vi "Test App Processes are Initialized.vi"(8 "error in (no error)":errorcluster, 11 "Rig Test In":refnum<class "Application Dev Test.lvclass">) -> (0 "error out":errorcluster, 3 "Rig Test Out":refnum<class "Application Dev Test.lvclass">)   [LabVIEW 2020, in "Application Dev Test.lvclass"]
uses:
  Application Dev Test.lvclass
  C:/Program Files (x86)/National Instruments/LabVIEW 2020/vi.lib/Astemes/LUnit/Test Case.lvclass
  source/Framework Test Suite/Mock Process/Mock Process.lvclass
  C:/Git/astemes-triarc-framework/source/Framework/Process/Process.lvclass
  source/Framework/Process/Process.lvclass/Process.ctl
  source/Framework/Application/Application.lvclass/Application.ctl
  <vilib>/Astemes/LUnit/Test Case.lvclass/Test Case.ctl
  source/Framework/Application/Private/Add Process to Map.vi
  source/Framework/Application/Private/Throw Error If Process Already in App.vi
  source/Framework/Process/Protected/Messaging/Send Message.vi
  source/Framework/Process/Public/Lifecycle/Get Lifecycle State.vi
  source/Framework/Process/Protected/SubVIs/Set Context.vi
  <vilib>/Astemes/LUnit/Palette/Fail.vi
  <vilib>/Astemes/LUnit/Palette/Pass.vi
  <vilib>/Astemes/LUnit/Set Assertion Type.vi
  source/Framework/Process/Protected/Messaging/Request Message.vi
  source/Framework/Process/Private/SubVIs/Wait for finish.vi
  source/Framework/Process/Private/SubVIs/Set Lifecycle State.vi
  source/Framework/Application/Public/Get Process.vi
  source/Framework/Process/Private/SubVIs/Handle Debug Data.vi
  <vilib>/Utility/error.llb/Clear Errors.vi
  source/Framework/Process/Public/Lifecycle/Leave Process Loop.vi
  <vilib>/Astemes/LUnit/Add test result.vi
  source/Framework/Process/Private/SubVIs/Enqueue Request Message.vi
  source/Framework/Application/Private/Retrieve Process from App.vi
  source/Framework/Application/Private/Parse Process Name.vi
  source/Framework/Application/Private/Get Process from Map.vi
  source/Framework/Logging/Log Debug.vi
  <vilib>/AdvancedString/1D String Array to Delimited String.vi
  <vilib>/Utility/High Resolution Relative Seconds.vi
  <vilib>/Astemes/LUnit/LUnit Record Assertion Result.vi
  <vilib>/AdvancedString/Delimited String to 1D String Array.vi
  <vilib>/Astemes/LUnit/LUnit Aggregate Assertion Results.vi
  <vilib>/Astemes/LUnit/Method Result/LUnit Merge Status.vi
  <vilib>/Astemes/LUnit/LUnit Concatenate result strings.vi
  source/Framework/Application/Application.lvclass
  <vilib>/Utility/error.llb/Error Cluster From Error Code.vi
  source/Framework/Process/Public/Read Name.vi
  source/Framework/Process/Private/SubVIs/Wait for Response Message.vi
  source/Framework/Process/Process.lvclass
  <vilib>/Astemes/LUnit/Test Case.lvclass
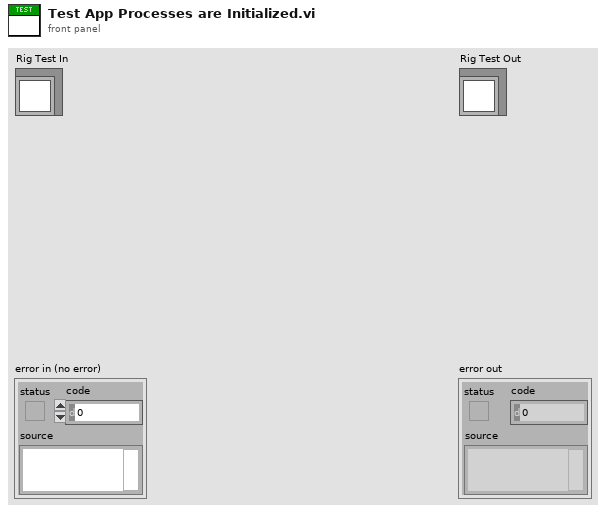
[diagram p1: front panel]
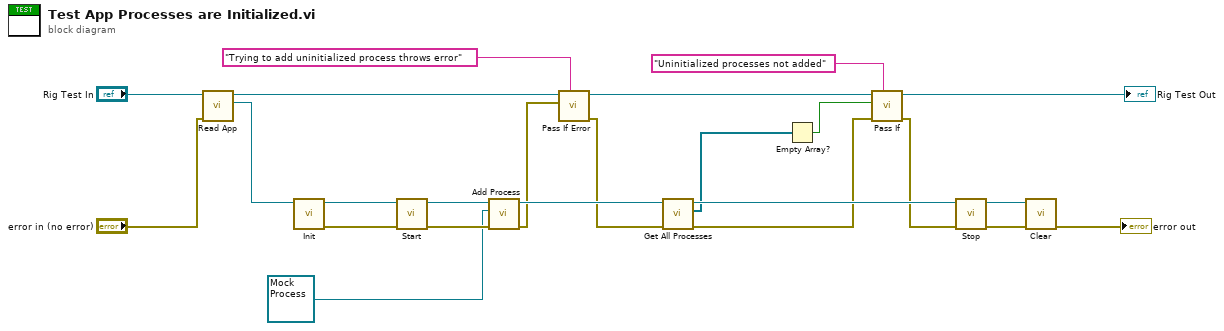
[diagram p0: block diagram]
diagram:
  n1 = call "Read App.vi"("error in (no error)"="error in (no error)", "Application Test In"="Rig Test In") -> ("App out"=w20:refnum<class "Application.lvclass">, "Application Test Out"=w14:refnum<class "Application Dev Test.lvclass">)  [unwired: 7 in, 1 out]
  n2 = call-dynamic "Init.vi"("Process In"=w20) -> ("error out"=w17:errorcluster, "Process Out"=w23:refnum<class "Application.lvclass">)  [unwired: 9 in]
  n3 = call "Start.vi"("error in (no error)"=w17, "Process In"=w23) -> ("error out"=w22:errorcluster, "Process Out"=w16:refnum<class "Application.lvclass">)  [unwired: 7 in, 1 out]
  n4 = call "Add Process.vi"("error in (no error)"=w22, "Process"=refnum<class "Mock Process.lvclass"> refnum ("Mock Process.lvclass"), "Application In"=w16) -> ("error out"=w5:errorcluster, "Application Out"=w19:refnum<class "Application.lvclass">)  [unwired: 7 in]
  n5 = call <vilib>:"Pass If Error.vi"("Description"="Trying to add uninitialized process throws error", "Assert error"=w5, "LUnit Test Case In"=w14) -> ("error out"=w4:errorcluster, "LUnit Test Case Out"=w6:refnum<class "Application Dev Test.lvclass">)  [unwired: 7 in]
  n6 = call "Get All Processes.vi"("error in (no error)"=w4, "Application In"=w19) -> ("error out"=w13:errorcluster, "App Processes"=w2:refnum<class "Process.lvclass">[], "Application Out"=w15:refnum<class "Application.lvclass">)  [unwired: 7 in]
  n7 = Empty Array?(array=w2) -> (empty?=w3:bool)
  n8 = call <vilib>:"Pass If.vi"("Description"="Uninitialized processes not added", "error in (no error)"=w13, "Pass?"=w3, "LUnit Test Case In"=w6) -> ("error out"=w11:errorcluster, "LUnit Test Case Out"=→"Rig Test Out":refnum<class "Application Dev Test.lvclass">)  [unwired: 6 in]
  n9 = call "Stop.vi"("error in (no error)"=w11, "Process In"=w15) -> ("error out"=w9:errorcluster, "Process Out"=w21:refnum<class "Application.lvclass">)  [unwired: 7 in, 1 out]
  n10 = call-dynamic "Clear.vi"("error in (no error)"=w9, "Application In"=w21) -> ("error out"=→"error out":errorcluster)  [unwired: 9 in]
